vi "Write String Constant Value.vi"(8 "error in":errorcluster, 10 "Python Function":string, 11 "Virtual Instrument in":refnum<class "Virtual Instrument.lvclass">) -> (0 "error out":errorcluster, 3 "Virtual Instrument out":refnum<class "Virtual Instrument.lvclass">)   [LabVIEW 2026, in "Virtual Instrument.lvclass"]
doc: "Replace the python function name constant by the corresponding function."
uses:
  Virtual Instrument.lvclass
  <vilib>/Utility/traverseref.llb/TRef TravTarget.ctl
  LabVIEW File/LabVIEW File.lvclass/LabVIEW File.ctl
  LabVIEW File/Read VI Reference.vi
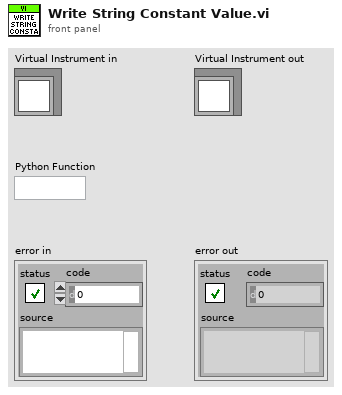
[diagram p1: front panel]
types:
  T1 = typedef "TRef TravTarget.ctl" = enum16{"FP", "BD", "Other"}
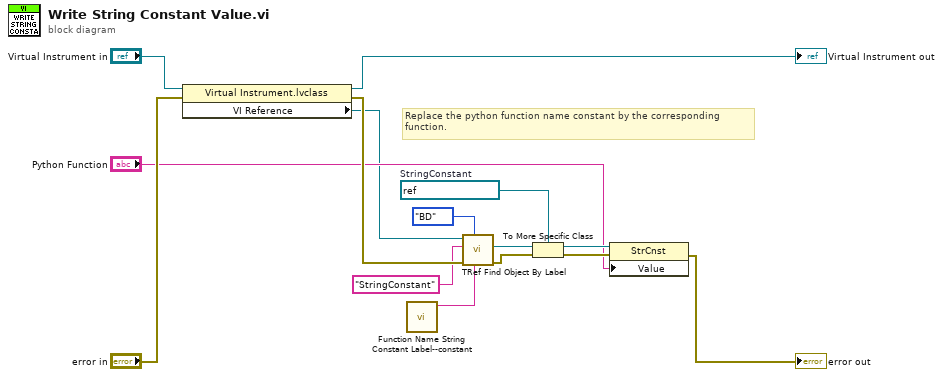
[diagram p0: block diagram]
diagram:
  w7 = refnum<vi> refnum  # StringConstant
  # "Replace the python function name constant by the corresponding\nfunction."
  n1 = property class="Virtual Instrument.lvclass"(reference="Virtual Instrument in", error in="error in") -> (reference out=→"Virtual Instrument out":refnum<class "Virtual Instrument.lvclass">, error out=w11:errorcluster, "VI Reference"=w1:refnum<vi>)
  n2 = call "Function Name String Constant Label--constant.vi"() -> ("Function Name String Constant Label"=w4:string)  [unwired: 11 in]
  n3 = call <vilib>:"TRef Find Object By Label.vi"("Label"=w4, "Traverse Target"=TRef_TravTarget."BD", "error in (no error)"=w11, "Class Name"="StringConstant", "VI Ref"=w1) -> ("error out"=w15:errorcluster, "Found Obj Ref"=w8:refnum<vi>)  [unwired: 3 in, 2 out]
  n4 = To More Specific Class(target class=w7, reference=w8, error in=w15) -> (specific class reference=w6:refnum<vi>, error out=w14:errorcluster)
  n5 = property class="StrCnst"(reference=w6, error in=w14, "Value"="Python Function") -> (error out=→"error out":errorcluster)  [unwired: 1 out]
